vi "Main.vi"() -> ()   [LabVIEW 2020]
doc: "Fall Detection main scaffold. While Loop and stop event are implemented. State_Machine call, polling timeout and main error chain remain manual tasks."
uses:
  Controls/State.ctl
panel:
  in  "内部log相对路径":path=path "Data/Main_native_samples.csv"
  in  "内部config相对路径":path=path "Config/P1_Runtime.ini"
  out "红色确认报警":bool
  out "黄色预警灯":bool
  out "蓝色提示":bool
  out "参数配置文件路径":path=path "C:/YOUXI/dazuoye/Config/P1_Runtime.ini"
  out "参数保存错误":errorcluster
  in  "报警倒计时时长（秒）":dbl=30.0 format="%#_13g"
  in  "疑似判定延时（秒）":dbl=5.0 format="%#_13g"
  out "日志写入失败":bool
  out "硬件初始化失败":bool
  out "硬件就绪":bool
  out "日志写入错误":errorcluster
  in  "手动求救":bool
  out "数字输出编码":dbl[](array[numeric])
  out "继电器控制信号":bool
  out "蜂鸣器控制信号":bool
  out "系统错误":errorcluster
  in  "硬件模式":bool
  out "光敏电压（伏）":dbl
  in  "停止":bool
  out "状态持续时间（秒）":dbl
  out "当前状态":T1
  in  "手动复位":bool
  in  "取消本次倒计时":bool
  in  "运动（仿真输入）":bool
  in  "倾斜（仿真输入）":bool
  out "剩余倒计时（秒）":dbl
  out "报警状态":bool
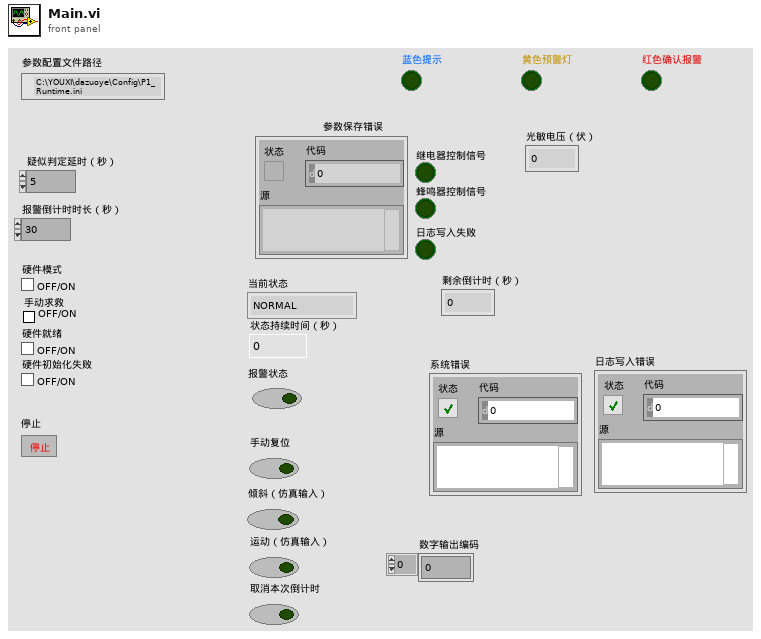
[diagram p1: front panel]
types:
  T1 = typedef "State.ctl" = enum16{"NORMAL", "SUSPECT", "COUNTDOWN", "ALARM", "RESET"}
  T2 = enum16{"open", "replace", "create", "open or create", "replace or create", "replace or create with confirmation"}
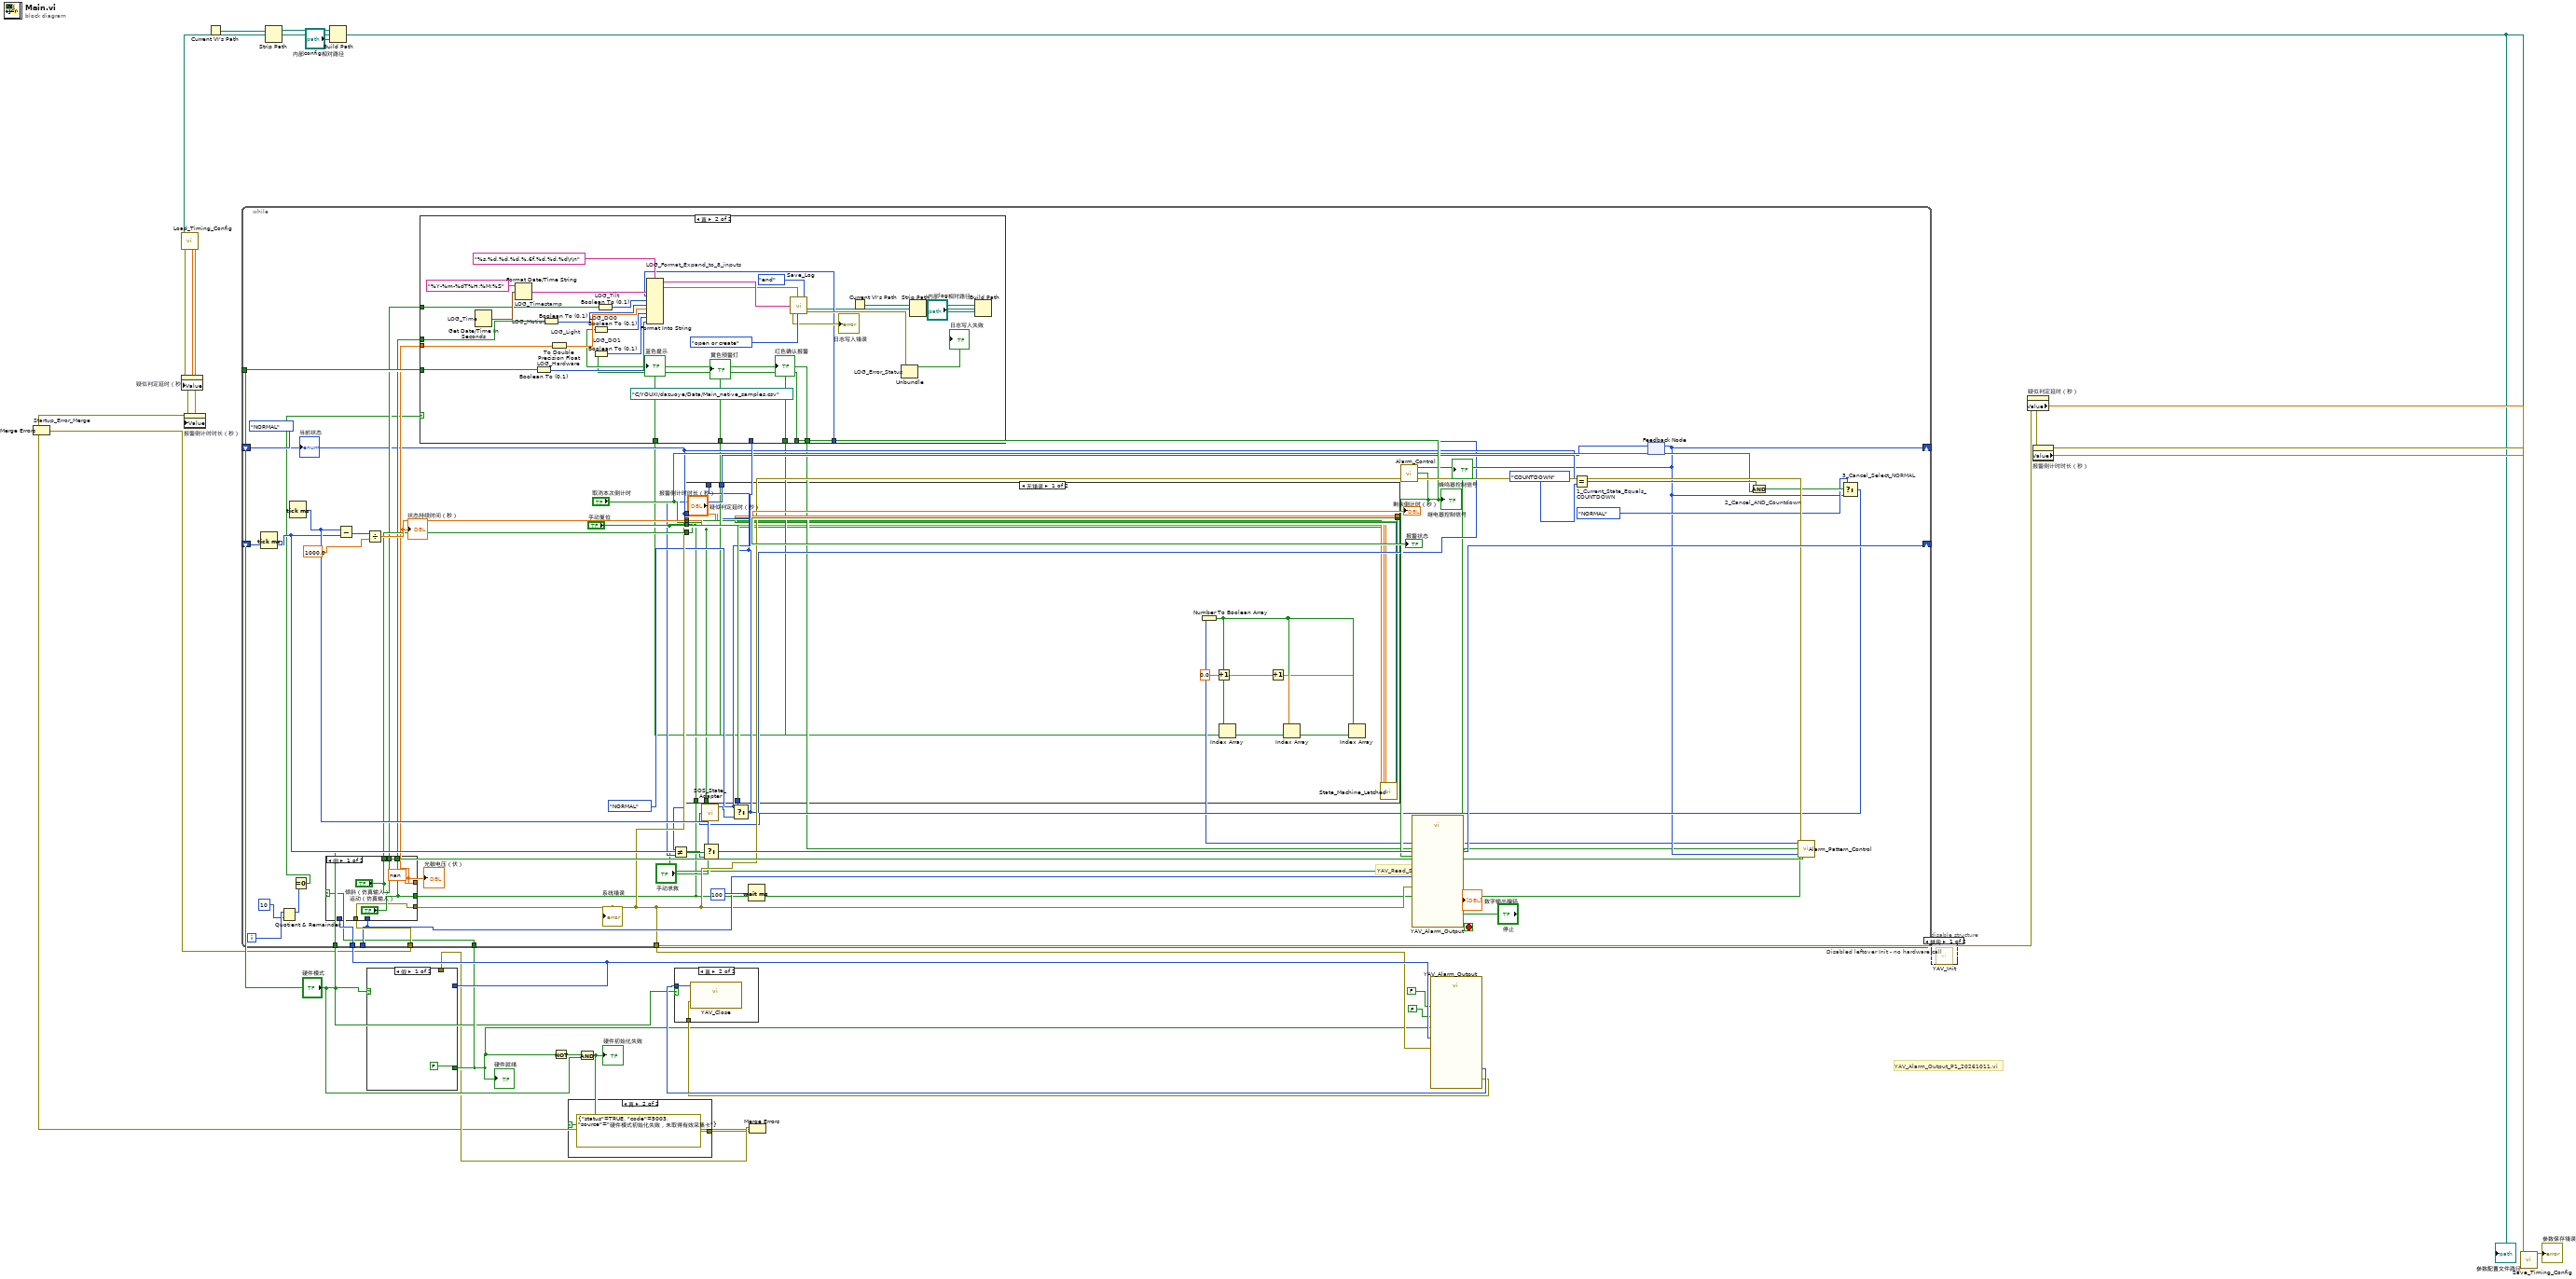
[diagram p0: block diagram]
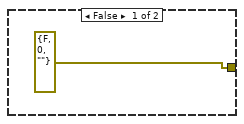
[diagram p2: hidden frame]
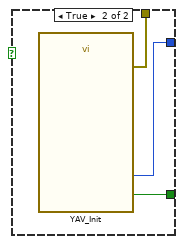
[diagram p5: hidden frame]
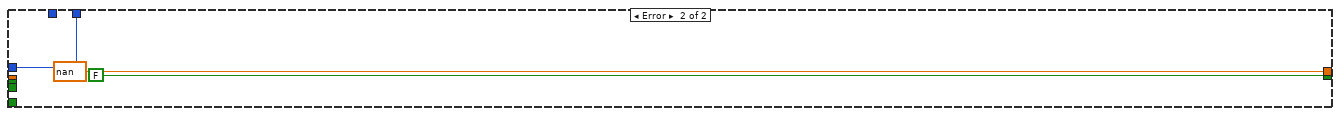
[diagram p7: hidden frame]
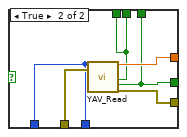
[diagram p8: hidden frame]
diagram:
  # "YAV_Alarm_Output_P1_20261011.vi"
  n1 = Current VI's Path() -> (path=w4:path)
  n2 = Tick Count (ms)() -> (millisecond timer value=w29:u32)
  n3 = Strip Path(path=w4) -> (stripped path=w3:path)  [unwired: 1 out]
  n4 = Build Path(base path=w3, name or relative path="内部config相对路径") -> (appended path=w1:path)
  "参数配置文件路径" <- w1
  n5 = call "Load_Timing_Config.vi"("INI File Path"=w1) -> ("INI Load Error"=w13:errorcluster, "Loaded Countdown (s)"=w14:dbl, "Loaded Suspect (s)"=w15:dbl)  [unwired: 8 in]
  n6 = property on="疑似判定延时（秒）" class="DigNum (严格)"(error in=w13, "Value"=w15) -> (error out=w12:errorcluster)  [unwired: 1 in, 1 out]
  n7 = property on="报警倒计时时长（秒）" class="DigNum (严格)"(error in=w12, "Value"=w14) -> (error out=w11:errorcluster)  [unwired: 1 in, 1 out]
  n8 = case shown="假" "硬件模式" {
    tunnel: [_ w34] -> w18
    tunnel: [_ w33] -> w28
    tunnel: [FALSE w32] -> w22
    frame False {
    }
    frame True {
      n9 = call "YAV_Init.vi"() -> ("Device ID"=w33:u32, "Hardware Valid"=w32:bool, "error out"=w34:errorcluster)  [unwired: 12 in, 1 out]
    }
  }
  "硬件就绪" <- w22
  n10 = Not(x=w22) -> (.not. x?=w21:bool)
  n11 = And(x=w21, y="硬件模式") -> (x .and. y?=w19:bool)
  "硬件初始化失败" <- w19
  n12 = case shown="真" w19 {
    tunnel: [errorcluster {"status"=FALSE, "code"=0, "source"=""} ("错误输出") errorcluster {"status"=TRUE, "code"=5003, "source"="硬件模式初始化失败，未取得有效采集卡"} ("错误输出")] -> w17
    frame False {
    }
    frame True {
    }
  }
  n13 = Merge Errors(w18, w17) -> (w16:errorcluster)
  n14 = Merge Errors "Startup_Error_Merge"(w16, w11) -> (w10:errorcluster)
  n15 = while {
    shift-right: [w50] -> _
    shift-left: State."NORMAL" ("Current State") -> [w53]
    shift-right: [w82] -> _
    shift-left: w29 -> [w83]
    tunnel: w28 -> [w76]
    tunnel: w10 -> [w75]
    tunnel: [w71] -> w24
    tunnel: "硬件模式" -> [w48]
    tunnel: [w72] -> _
    tunnel: "硬件模式" -> [w67]
    tunnel: w22 -> [w47]
    i -> [w62]
    stop <- "停止" stop-if-true
    w65 = State."NORMAL" ("Current State")
    # "YAV_Read_Sprint.vi"
    n16 = Quotient & Remainder(x=w62, y=10) -> (x-y*floor(x/y)=w60:i32)  [unwired: 1 out]
    n17 = Tick Count (ms)() -> (millisecond timer value=w84:u32)
    n18 = Equal To 0?(x=w60) -> (x = 0?=w59:bool)
    n19 = case shown="假" w47 {
      tunnel: w76 -> [_ w139]
      tunnel: w75 -> [w133 w142]
      tunnel: [w133 w141] -> w71
      tunnel: [nan ("Light Voltage (V)") w140] -> w66
      tunnel: ["倾斜（仿真输入）" w137] -> w74
      tunnel: ["运动（仿真输入）" w138] -> w37
      tunnel: [_ w139] -> w72
      tunnel: ["运动（仿真输入）" w138] -> w64
      tunnel: ["倾斜（仿真输入）" w137] -> w63
      frame False {
      }
      frame True {
        n20 = call "YAV_Read.vi"("Device ID"=w139, "error in"=w142) -> ("Light Voltage (V)"=w140:dbl, "Tilt"=w137:bool, "Motion"=w138:bool, "error out"=w141:errorcluster)  [unwired: 12 in, 2 out]
      }
    }
    "光敏电压（伏）" <- w66
    "系统错误" <- w71
    n21 = Subtract(x=w84, y=w83) -> (x-y=w88:u32)
    n22 = Divide(x=w88, y=1000.0) -> (x/y=w87:dbl)
    "状态持续时间（秒）" <- w87
    n23 = Wait (ms)(milliseconds to wait=100) -> ()  [unwired: 1 out]
    n24 = Increment(x=0.0) -> (x+1=w43:dbl)
    n25 = Increment(x=w43) -> (x+1=w41:dbl)
    n26 = Equal? "1_Current_State_Equals_COUNTDOWN"(x=w53, y=State."COUNTDOWN" ("Current State")) -> (x = y?=w58:bool)
    n27 = feedback #1() -> (w50:T1)  [unwired: 1 in]
    n28 = call "Alarm_Control.vi"("State"=w50, "error in"=w71) -> ("DO1 Software"=w68:bool)  [unwired: 3 in, 2 out]
    "继电器控制信号" <- w68
    n29 = And "2_Cancel_AND_Countdown"(x=w58, y="取消本次倒计时") -> (x .and. y?=w57:bool)
    n30 = call "Alarm_Pattern_Control.vi"("error in (no error)"=w71, "Tilt"=w74, "Motion"=w37, "State Value"=w50) -> ("Warning Code"=w45:u32, "DO0 Pattern"=w46:bool)  [unwired: 1 in, 1 out]
    "蜂鸣器控制信号" <- w46
    n31 = Number To Boolean Array(number=w45) -> (Boolean array=w42:bool[])
    n32 = Index Array(array=w42) -> (element=w40:bool)  [unwired: 1 in]
    n33 = Index Array(array=w42, index=w43) -> (element=w39:bool)
    n34 = Index Array(array=w42, index=w41) -> (element=w38:bool)
    n35 = call "YAV_Alarm_Output.vi"("DO0"=w46, "DO1"=w68, "错误输入（无错误）"=w71, "ID"=w72, "Hardware Enable"=w48) -> ("Encoded Buffer"=→"数字输出编码":dbl[])  [unwired: 2 out]
    n36 = Select "3_Cancel_Select_NORMAL"(t=State."NORMAL" ("Current State"), s=w57, f=w50) -> (s? t:f=w52:T1)
    n37 = call "SOS_State_Adapter.vi"("Current State"=w52, "SOS Pressed"="手动求救") -> ("State To Machine"=w69:T1)  [unwired: 2 in, 3 out]
    n38 = Select(t=w65, s="手动复位", f=w69) -> (s? t:f=w49:T1)
    n39 = case shown="真" w59 {
      tunnel: w46 -> [_ w103]
      tunnel: w68 -> [_ w102]
      tunnel: w67 -> [_ w101]
      tunnel: w66 -> [_ w100]
      tunnel: w65 -> [_ _]
      tunnel: w64 -> [_ w99]
      tunnel: w63 -> [_ w98]
      tunnel: w49 -> [_ w97]
      tunnel: w40 -> [_ w95]
      tunnel: w39 -> [_ w94]
      tunnel: w38 -> [_ w93]
      frame False {
      }
      frame True {
        (unwired) path "C:/YOUXI/dazuoye/Data/Main_native_samples.csv" ("日志文件路径")
        n40 = Get Date/Time In Seconds "LOG_Time"() -> (seconds since 1Jan1904=w118:timestamp)
        n41 = Format Date/Time String "LOG_Timestamp"(time format string (%c)="%Y-%m-%dT%H:%M:%S" ("时间格式字符串(%c)"), seconds (now)=w118) -> (date/time string=w115:string)  [unwired: 1 in]
        n42 = Boolean To (0,1) "LOG_Hardware"(Boolean=w101) -> (0, 1=w105:i16)
        n43 = Boolean To (0,1) "LOG_Motion"(Boolean=w99) -> (0, 1=w108:i16)
        n44 = To Double Precision Float "LOG_Light"(number=w100) -> (double precision float=w104:dbl)
        n45 = Boolean To (0,1) "LOG_DO0"(Boolean=w103) -> (0, 1=w107:i16)
        n46 = Boolean To (0,1) "LOG_DO1"(Boolean=w102) -> (0, 1=w106:i16)
        n47 = Boolean To (0,1) "LOG_Tilt"(Boolean=w98) -> (0, 1=w109:i16)
        n48 = Format Into String "LOG_Format_Expand_to_8_inputs"(format string="%s,%d,%d,%d,%.6f,%d,%d,%d\r\n" ("格式字符串"), w115, w97, w109, w108, w104, w107, w106, w105) -> (resulting string=w114:string, error out=w113:errorcluster)  [unwired: 2 in]
        n49 = Current VI's Path() -> (path=w92:path)
        n50 = Strip Path(path=w92) -> (stripped path=w91:path)  [unwired: 1 out]
        n51 = Build Path(base path=w91, name or relative path="内部log相对路径") -> (appended path=w89:path)
        n52 = call "Save_Log.vi"("日志文件路径"=w89, "错误输入"=w113, "日志记录行"=w114, "打开或新建"=T2."open or create", "写入位置（末尾）"=enum16{"start", "end", "current"}."end") -> ("错误输出"=w110:errorcluster)  [unwired: 2 in]
        "日志写入错误" <- w110
        n53 = Unbundle "LOG_Error_Status"(w110) -> ("status"=→"日志写入失败":bool)  [unwired: 2 out]
        "蓝色提示" <- w95
        "黄色预警灯" <- w94
        "红色确认报警" <- w93
      }
    }
    n54 = case shown="无错误" w71 {
      tunnel: w87 -> [w129 _]
      tunnel: w53 -> [_ w132]
      tunnel: [w128 w132] -> w51
      tunnel: [w127 FALSE ("Alarm")] -> w81
      tunnel: [w126 nan ("Countdown")] -> w80
      tunnel: "取消本次倒计时" -> [w125 _]
      tunnel: "手动复位" -> [w122 _]
      tunnel: w74 -> [w124 _]
      tunnel: w37 -> [w123 _]
      tunnel: w49 -> [_ _]
      tunnel: [w122 _] -> _
      tunnel: w49 -> [w121 _]
      frame No Error {
        n55 = call "State_Machine_Latched.vi"("Current State"=w121, "Tilt"=w124, "Motion"=w123, "State Elapsed (s)"=w129, "Cancel"=w125, "Reset"=w122, "Suspect Delay (s)"="疑似判定延时（秒）", "Countdown Duration (s)"="报警倒计时时长（秒）") -> ("Next State"=w128:T1, "Countdown"=w126:dbl, "Alarm"=w127:bool)  [unwired: 16 in, 1 out]
      }
      frame Error {
      }
    }
    "报警状态" <- w81
    "剩余倒计时（秒）" <- w80
    n56 = Not Equal?(x=w53, y=w51) -> (x != y?=w85:bool)
    n57 = Select(t=w84, s=w85, f=w83) -> (s? t:f=w82:u32)
    n58 = feedback-in #1(w51) -> ()
    "当前状态" <- w53
  }
  n59 = call "YAV_Alarm_Output.vi"("DO0"=FALSE, "DO1"=FALSE, "错误输入（无错误）"=w24, "ID"=w28, "Hardware Enable"=w22) -> ("错误输出"=w23:errorcluster, "ID 2"=w27:u32)  [unwired: 1 out]
  n60 = case shown="真" "硬件模式" {
    tunnel: w27 -> [_ w144]
    tunnel: w23 -> [_ w143]
    frame False {
    }
    frame True {
      n61 = call "YAV_Close.vi"("error in"=w143, "Device ID"=w144) -> ()  [unwired: 9 in, 1 out]
    }
  }
  n62 = disable-structure "Disabled leftover Init - no hardware call" shown="禁用" {
    frame Disabled {
      n63 = call "YAV_Init.vi"() -> ()  [unwired: 12 in, 4 out]
    }
    frame Enabled {
    }
  }
  n64 = property on="疑似判定延时（秒）" class="DigNum (严格)"(error in=w24) -> (error out=w8:errorcluster, "Value"=w6:dbl)  [unwired: 1 in, 1 out]
  n65 = property on="报警倒计时时长（秒）" class="DigNum (严格)"(error in=w8) -> (error out=w7:errorcluster, "Value"=w5:dbl)  [unwired: 1 in, 1 out]
  n66 = call "Save_Timing_Config.vi"("INI Save Error In"=w7, "Save Countdown (s)"=w5, "Save Suspect (s)"=w6, "Save INI File Path"=w1) -> ("INI Save Error"=→"参数保存错误":errorcluster)  [unwired: 7 in]
